vi "ERW-IoT Telemetry Draft.vi"() -> ()   [LabVIEW 2026]
panel:
  out "Latest Telemetry":string
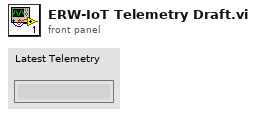
[diagram p1: front panel]
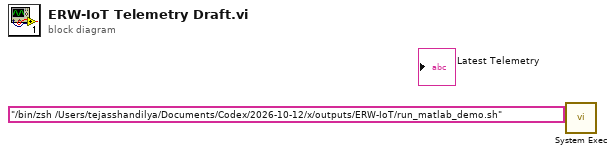
[diagram p0: block diagram]
diagram:
  (unwired) "/bin/zsh /Users/tejasshandilya/Documents/Codex/2026-10-12/x/outputs/ERW-IoT/run_matlab_demo.sh"
  n1 = call <vilib>:"System Exec.vi"() -> ()  [unwired: 8 in, 4 out]
